vi "Test - Prepare Case Folder.vi"(8 "error in (no error)":errorcluster, 9 "Case Name":string, 10 "Work Folder":path, 11 "Source Folder":path) -> (0 "error out":errorcluster, 3 "Case Folder":path)   [LabVIEW 2024]
doc: "Creates a new, empty case folder <Work Folder>\\<Case Name> <date-time> and copies every *.ini file of Source Folder into it. Tests work on that copy, so the source data is never changed and every run starts from the same files. Returns the case folder.\n\nGenerated by: Claude"
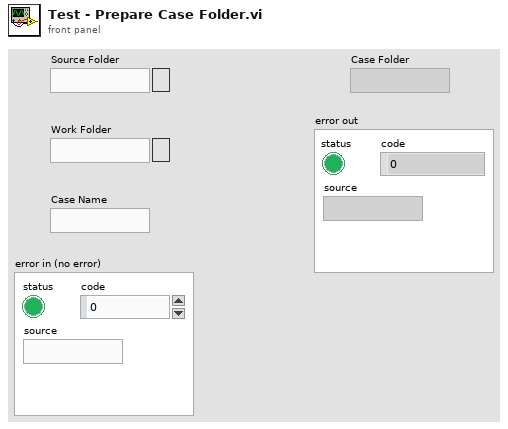
[diagram p1: front panel]
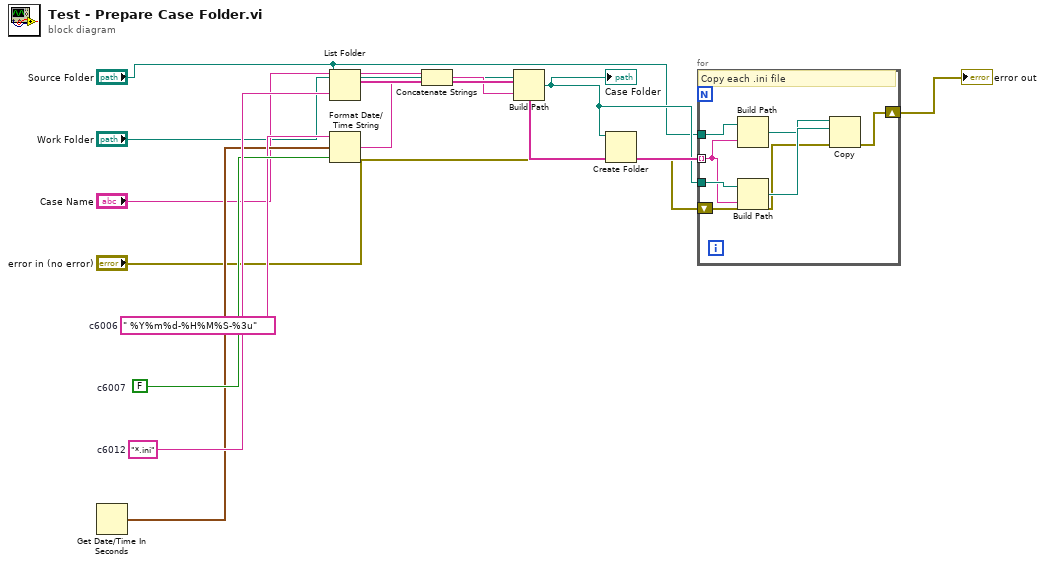
[diagram p0: block diagram]
diagram:
  w12 = "*.ini"  # c6012
  w7 = FALSE  # c6007
  w6 = " %Y%m%d-%H%M%S-%3u"  # c6006
  n1 = Get Date/Time In Seconds() -> (seconds since 1Jan1904=w5:timestamp)
  n2 = List Folder(path="Source Folder", pattern=w12) -> (filenames=w13:string[])  [unwired: 2 in, 3 out]
  n3 = Format Date/Time String(time format string (%c)=w6, seconds (now)=w5, UTC format=w7) -> (date/time string=w8:string)
  n4 = Concatenate Strings("Case Name", w8) -> (w9:string)
  n5 = Build Path(base path="Work Folder", name or relative path=w9) -> (appended path=w10:path)
  "Case Folder" <- w10
  n6 = Create Folder(path (use dialog)=w10, error in="error in (no error)") -> (error out=w11:errorcluster)  [unwired: 1 in, 2 out]
  n7 = for {
    tunnel: "Source Folder" -> [w16]
    tunnel: w13 -> [w15] mode=indexing
    tunnel: w10 -> [w17]
    shift-right: [w19] -> w14
    shift-left: w11 -> [w18]
    # "Copy each .ini file"
    n8 = Build Path(base path=w16, name or relative path=w15) -> (appended path=w20:path)
    n9 = Build Path(base path=w17, name or relative path=w15) -> (appended path=w21:path)
    n10 = Copy(8:w18, 10:w21, 11:w20) -> (0:w19:errorcluster)  [unwired: 2 in, 2 out]
  }
  "error out" <- w14
